vi "C_Check_Return.vi"(8 "error in (no error)":errorcluster, 10 "function name":string, 11 "function return":i32) -> (0 "error out":errorcluster, 2 "length":i32, 3 "ok":bool)   [LabVIEW 2021, in "CANsub_C.lvlib"]
doc: "Converts a negative return value of a libcansub_codec function into a LabVIEW error: code 5100 - return value (5101 buffer too small, 5102 invalid input, 5103 no solution, 5104 state not initialised). An incoming error is kept first."
uses:
  CANsub_C.lvlib
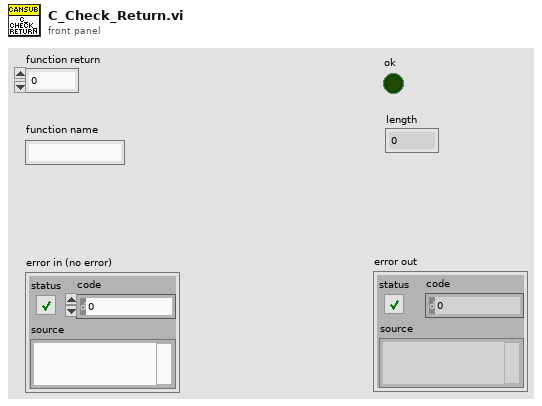
[diagram p1: front panel]
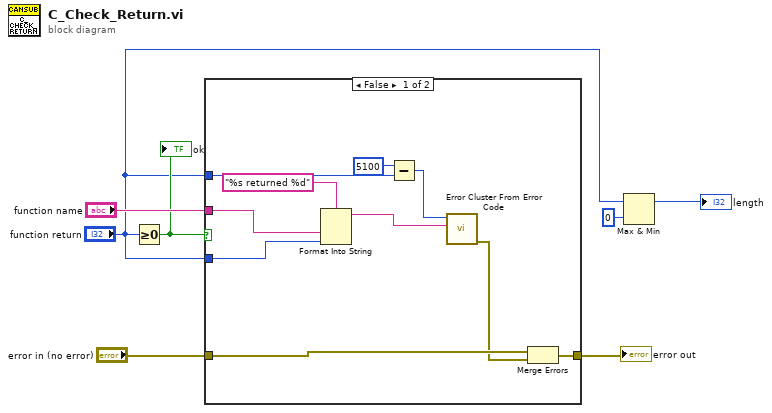
[diagram p0: block diagram]
diagram:
  n1 = Greater Or Equal To 0?(x="function return") -> (x >= 0?=w4:bool)
  "ok" <- w4
  n2 = case shown="False" w4 {
    tunnel: [w11 w18] -> w7
    tunnel: "error in (no error)" -> [w10 w18]
    tunnel: "function name" -> [w16 _]
    tunnel: "function return" -> [w15 _]
    tunnel: "function return" -> [w13 _]
    frame False {
      n3 = Format Into String(format string="%s returned %d", w16, w15) -> (resulting string=w12:string)  [unwired: 2 in, 1 out]
      n4 = Subtract(x=5100, y=w13) -> (x-y=w8:i32)
      n5 = call <vilib>:"Error Cluster From Error Code.vi"("error message (\"\")"=w12, "error code (0)"=w8) -> ("error out"=w9:errorcluster)  [unwired: 7 in]
      n6 = Merge Errors(w10, w9) -> (w11:errorcluster)
    }
    frame True {
    }
  }
  "error out" <- w7
  n7 = Max & Min(x="function return", y=0) -> (max(x,y)=→"length":i32)  [unwired: 1 out]
